vi "Main.vi"(0 "Proto File Path":path[](array[path]), 1 "Generated Library Name":string, 2 "Generate Server or Client?":enum16{"gRPC Server", "gRPC Client", "Both"}(ring), 3 "type of dialog (OK msg:1)":T1=1 items=["no dialog", "OK message", "continue or stop message", "OK message + warnings", "continue/stop + warnings"], 5 "Import Paths":path[](array[path]), 7 "Prototype Library":path, 9 "Target Project":path, 11 "Target Name":string, 12 "Library Suffix":string caption="Generated Library Suffix (\"_server\" / \"_client\" will be added by default)") -> (15 "error out":errorcluster)   [LabVIEW 2019, in "gRPC Template Creation Utility.lvlib"]
uses:
  gRPC Template Creation Utility.lvlib
  <vilib>/Utility/error.llb/DialogType.ctl
  TypeDefs/Project Settings.ctl
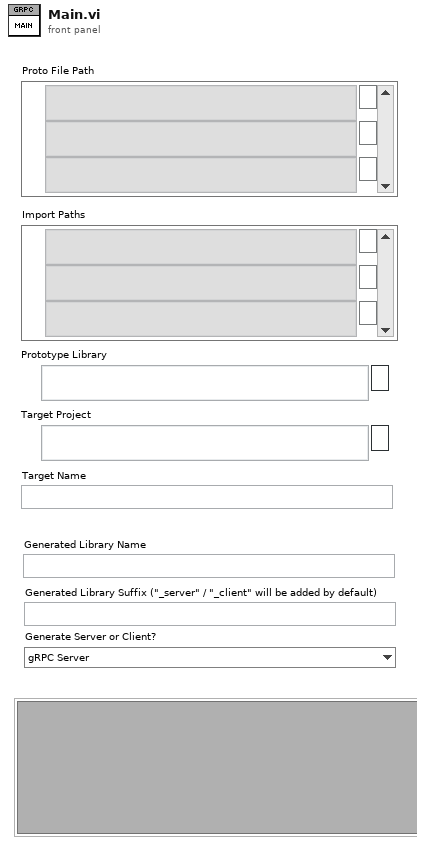
[diagram p1: front panel]
types:
  T1 = typedef "DialogType.ctl" = u16
  T2 = typedef "gRPC Template Creation Utility.lvlib/RPC Method Parameters.ctl" = cluster{"RPC Method Name":string, "Request Metadata Name":string, "Response Metadata Name":string, "Client Streaming":bool, "Server Streaming":bool}
  T3 = typedef "gRPC Template Creation Utility.lvlib/Enum Metadata (Scripting).ctl" = cluster{"Version":i32, "Name":string, "Type Url":string, "Enum Values":string, "Allow Alias":bool}
  T4 = typedef "gRPC Template Creation Utility.lvlib/Message Metadata (Scripting).ctl" = cluster{"Version":i32, "Name":string, "Type Url":string, "Elements":T5[], "Has Oneof":bool}
  T5 = typedef "gRPC Template Creation Utility.lvlib/Message Element Metadata (Scripting).ctl" = cluster{"Field Name":string, "Embedded Message Name":string, "Protobuf Index":i32, "MessageElementType":T6, "Repeated":bool, "Is in Oneof":bool, "Oneof Container Name":string}
  T6 = typedef "gRPC Template Creation Utility.lvlib/Message Element Type.ctl" = enum32{"Int32Value", "FloatValue", "DoubleValue", "BoolValue", "StringValue", "MessageValue", "Int64Value", "UInt32Value", "UInt64Value", "EnumValue", "Bytes", "Fixed64", "Fixed32", "SFixed64", "SFixed32", "SInt64", "SInt32"}
  T7 = typedef "gRPC Template Creation Utility.lvlib/Project Settings.ctl" = cluster{"Target Project Path":path, "Target Name":string, "Server Name":string, "Library Path":path}
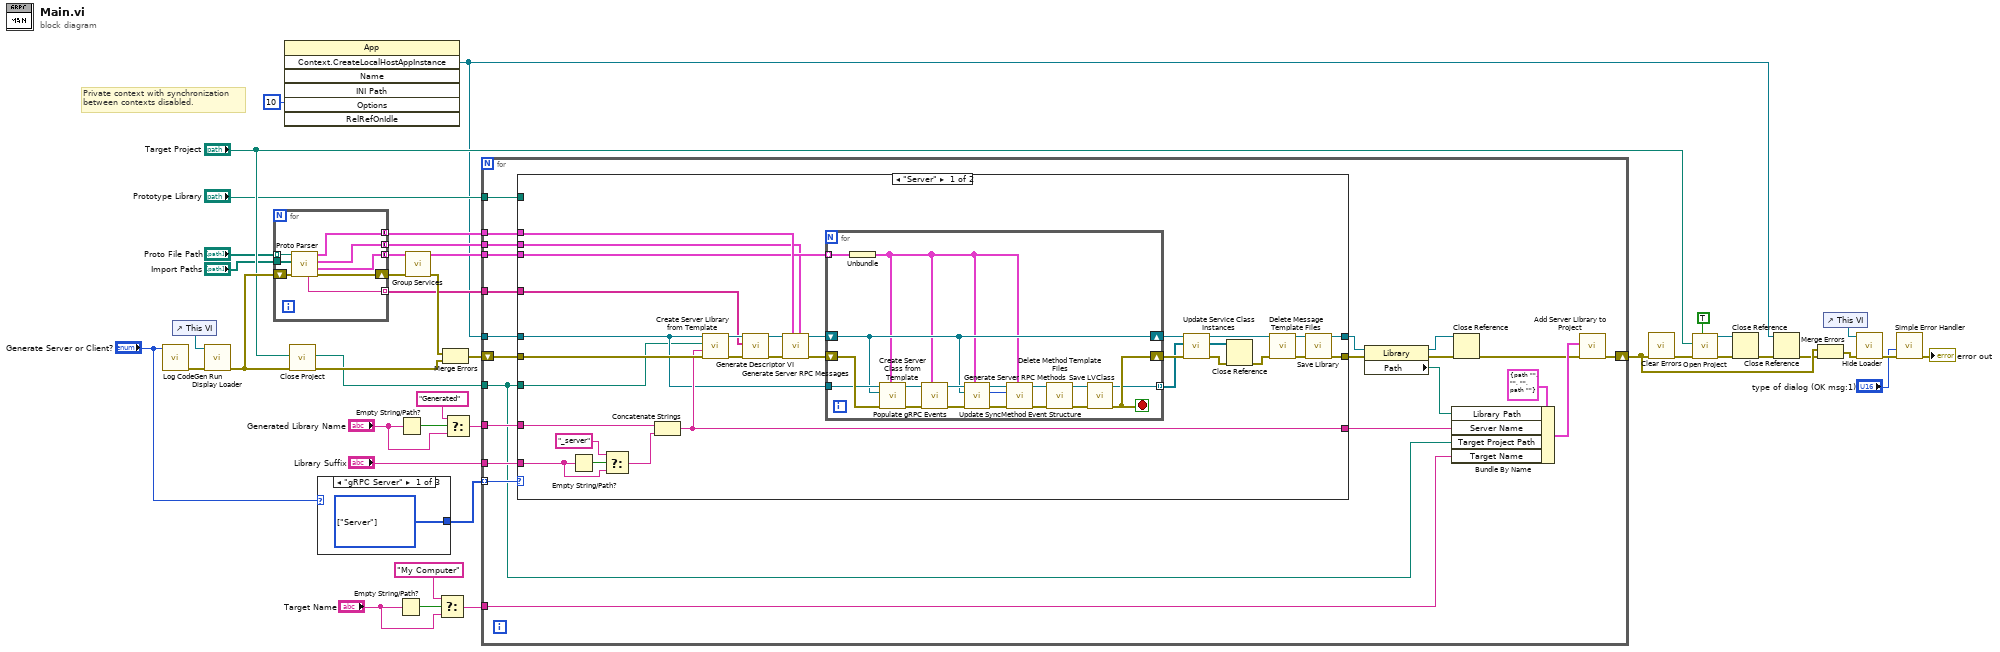
[diagram p0: block diagram]
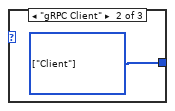
[diagram p2: hidden frame]
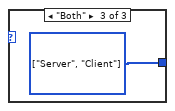
[diagram p3: hidden frame]
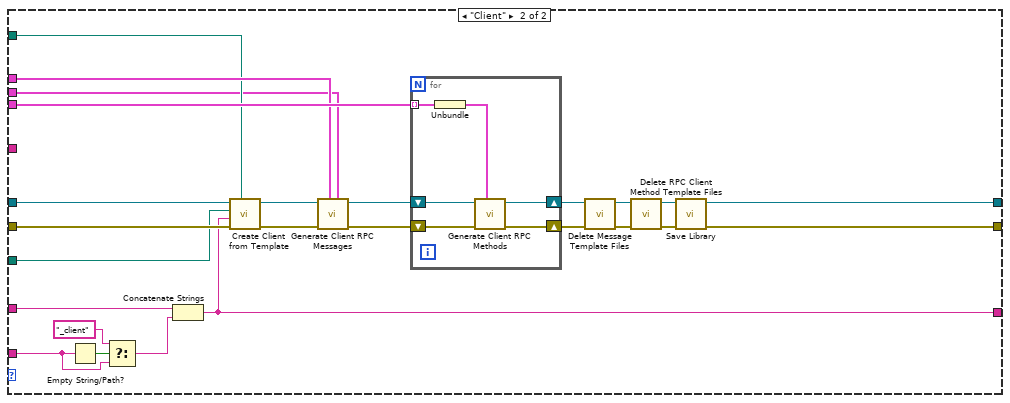
[diagram p4: hidden frame]
diagram:
  # "Private context with synchronization\nbetween contexts disabled."
  n1 = call "Log CodeGen Run.vi"("To Generate"="Generate Server or Client?") -> ("error out"=w8:errorcluster)  [unwired: 10 in]
  n2 = control-ref of="This VI"() -> (w7:refnum<vi>)
  n3 = call "Display Loader.vi"("error in (no error)"=w8, "VI in"=w7) -> ("error out"=w35:errorcluster)  [unwired: 9 in]
  n4 = for {
    tunnel: [w45] -> w37 mode=concatenating
    tunnel: [w49] -> w16 mode=concatenating
    shift-right: [w50] -> w18
    shift-left: w35 -> [w48]
    tunnel: "Proto File Path" -> [w47] mode=indexing
    tunnel: "Import Paths" -> [w46]
    tunnel: [w44] -> w11 mode=concatenating
    tunnel: [w43] -> w10 mode=indexing
    n5 = call "Proto Parser.vi"("error in (no error)"=w48, "Import Paths"=w46, ".proto file path"=w47) -> ("error out"=w50:errorcluster, "gRPC Method Parameters"=w49:T2[], "gRPC Enum Parameters"=w44:T3[], "gRPC Message Parameters"=w45:T4[], "Serialized Proto"=w43:string)  [unwired: 4 in]
  }
  n6 = invoke class="App" method="Context.CreateLocalHostAppInstance"("Options"=10) -> ("Create Context"=w3:refnum<vi>)  [unwired: 6 in, 6 out]
  n7 = call "Close Project.vi"("error in (no error)"=w35, "Project Path in"="Target Project") -> ("error out"=w39:errorcluster, "Project Path out"=w33:path)  [unwired: 8 in]
  n8 = case shown="\"gRPC Server\"" "Generate Server or Client?" {
    tunnel: [w51 w52 w53] -> w27
    frame "gRPC Server" {
      w51 = enum16{"Server", "Client"}[] [enum."Server"] items=["Server", "Client"]
    }
    frame "gRPC Client" {
      w52 = enum16{"Server", "Client"}[] [enum."Client"] items=["Server", "Client"]
    }
    frame "Both" {
      w53 = enum16{"Server", "Client"}[] [enum."Server", enum."Client"] items=["Server", "Client"]
    }
  }
  n9 = Empty String/Path?(string/path="Target Name") -> (empty?=w30:bool)
  n10 = Empty String/Path?(string/path="Generated Library Name") -> (empty?=w42:bool)
  n11 = call "Group Services.vi"("error in"=w18, "gRPC Method Parameters"=w16) -> ("error out"=w17:errorcluster, "Service Methods"=w15:cluster{"gRPC Method Parameters":T2[]}[])  [unwired: 8 in]
  n12 = Select(t="My Computer" ("Path"), s=w30, f="Target Name") -> (s? t:f=w28:string)
  n13 = Merge Errors(w17, w39) -> (w38:errorcluster)
  n14 = Select(t="Generated" ("Path"), s=w42, f="Generated Library Name") -> (s? t:f=w32:string)
  n15 = for {
    tunnel: w37 -> [w74]
    tunnel: w15 -> [w73]
    tunnel: w33 -> [w58]
    tunnel: w32 -> [w66]
    tunnel: w28 -> [w57]
    tunnel: w3 -> [w64]
    shift-right: [w61] -> w20
    shift-left: w38 -> [w75]
    tunnel: w27 -> [w60] mode=indexing
    tunnel: "Library Suffix" -> [w59]
    tunnel: "Prototype Library" -> [w56]
    tunnel: w11 -> [w55]
    tunnel: w10 -> [w54]
    n16 = case shown="\"Server\"" w60 {
      tunnel: w75 -> [w105 w148]
      tunnel: w74 -> [w104 w139]
      tunnel: w73 -> [w103 w147]
      tunnel: [w102 w146] -> w72
      tunnel: [w90 w138] -> w70
      tunnel: w66 -> [w101 w145]
      tunnel: [w100 w144] -> w65
      tunnel: w64 -> [w99 w143]
      tunnel: w58 -> [w98 w142]
      tunnel: w59 -> [w91 w133]
      tunnel: w56 -> [_ w131]
      tunnel: w55 -> [w83 w126]
      tunnel: w54 -> [w84 _]
      frame "Server" {
        n17 = Empty String/Path?(string/path=w91) -> (empty?=w94:bool)
        n18 = Select(t="_server" ("string"), s=w94, f=w91) -> (s? t:f=w92:string)
        n19 = Concatenate Strings(w101, w92) -> (w100:string)
        n20 = call "Create Server Library from Template.vi"("error in (no error)"=w105, "Generated Server Name"=w100, "Target Project Path"=w98, "Application ref in"=w99) -> ("error out"=w88:errorcluster, "Server library"=w86:refnum<vi>)  [unwired: 6 in]
        n21 = call "Generate Descriptor VI.vi"("error in (no error)"=w88, "Descriptor Strings"=w84, "Library in"=w86) -> ("error out"=w87:errorcluster, "Library out"=w85:refnum<vi>)  [unwired: 7 in]
        n22 = call "Generate Server RPC Messages.vi"("Enum Metadata"=w83, "Messages Metadata"=w104, "error in (no error)"=w87, "Library in"=w85) -> ("error out"=w89:errorcluster, "Library out"=w97:refnum<vi>)  [unwired: 6 in]
        n23 = for {
          tunnel: w103 -> [w121] mode=indexing
          shift-right: [w116] -> w81
          shift-left: w97 -> [w116]
          tunnel: w99 -> [w122]
          shift-right: [w108] -> w82
          shift-left: w89 -> [w123]
          tunnel: [w107] -> w79 mode=indexing
          stop <- w108 stop-if-true
          n24 = Unbundle(w121) -> ("gRPC Method Parameters"=w110:T2[])
          n25 = call "Create Server Class from Template.vi"("gRPC Method Parameters"=w110, "error in (no error)"=w123, "Library"=w116, "Application ref in"=w122) -> ("error out"=w119:errorcluster, "LVClassLibrary"=w120:refnum<vi>)  [unwired: 5 in, 1 out]
          n26 = call "Populate gRPC Events.vi"("RPC Method Parameters"=w110, "error in (no error)"=w119, "Server class in"=w120) -> ("error out"=w117:errorcluster, "Server class out"=w118:refnum<vi>)  [unwired: 7 in]
          n27 = call "Generate Server RPC Methods.vi"("RPC Method Parameters"=w110, "error in (no error)"=w117, "Library"=w116, "Server class in"=w118) -> ("error out"=w113:errorcluster, "Newly created methods count"=w109:i64, "Server class out"=w115:refnum<vi>)  [unwired: 5 in]
          n28 = call "Update SyncMethod Event Structure.vi"("gRPC Method Parameters"=w110, "error in (no error)"=w113, "Newly created methods count"=w109, "Server class in"=w115) -> ("error out"=w112:errorcluster, "Server class out"=w114:refnum<vi>)  [unwired: 6 in]
          n29 = call "Delete Method Template Files.vi"("error in (no error)"=w112, "LVClassLibrary in"=w114) -> ("error out"=w106:errorcluster, "LVClassLibrary out"=w111:refnum<vi>)  [unwired: 8 in]
          n30 = call "Save LVClass.vi"("error in (no error)"=w106, "LVClassLibrary in"=w111) -> ("error out"=w108:errorcluster, "LVClassLibrary out"=w107:refnum<vi>)  [unwired: 8 in]
        }
        n31 = call "Update Service Class Instances.vi"("error in (no error)"=w82, "service classes in"=w79, "server library in"=w81) -> ("error out"=w78:errorcluster, "service classes out"=w76:refnum<vi>[], "server library out"=w80:refnum<vi>)  [unwired: 6 in]
        n32 = Close Reference(reference=w76, error in (no error)=w78) -> (error out=w77:errorcluster)
        n33 = call "Delete Message Template Files.vi"("error in (no error)"=w77, "library in"=w80) -> ("error out"=w96:errorcluster, "library out"=w95:refnum<vi>)  [unwired: 8 in]
        n34 = call "Save Library.vi"("error in (no error)"=w96, "Library in"=w95) -> ("error out"=w90:errorcluster, "Library out"=w102:refnum<vi>)  [unwired: 8 in]
      }
      frame "Client" {
        n35 = Empty String/Path?(string/path=w133) -> (empty?=w135:bool)
        n36 = Select(t="_client" ("string"), s=w135, f=w133) -> (s? t:f=w132:string)
        n37 = Concatenate Strings(w145, w132) -> (w144:string)
        n38 = call "Create Client from Template.vi"("Template Library"=w131, "error in (no error)"=w148, "Generated Server Name"=w144, "Target Project Path"=w142, "Application ref in"=w143) -> ("error out"=w141:errorcluster, "Client library out"=w140:refnum<vi>)  [unwired: 5 in]
        n39 = call "Generate Client RPC Messages.vi"("Enum Metadata"=w126, "Messages Metadata"=w139, "error in (no error)"=w141, "Library in"=w140) -> ("error out"=w125:errorcluster, "Library out"=w124:refnum<vi>)  [unwired: 6 in]
        n40 = for {
          tunnel: w147 -> [w154] mode=indexing
          shift-right: [w149] -> w129
          shift-left: w124 -> [w151]
          shift-right: [w150] -> w130
          shift-left: w125 -> [w152]
          n41 = Unbundle(w154) -> ("gRPC Method Parameters"=w153:T2[])
          n42 = call "Generate Client RPC Methods.vi"("rpc method parameters"=w153, "error in (no error)"=w152, "library in"=w151) -> ("error out"=w150:errorcluster, "library out"=w149:refnum<vi>)  [unwired: 7 in]
        }
        n43 = call "Delete Message Template Files.vi"("error in (no error)"=w130, "library in"=w129) -> ("error out"=w127:errorcluster, "library out"=w128:refnum<vi>)  [unwired: 8 in]
        n44 = call "Delete RPC Client Method Template Files.vi"("error in (no error)"=w127, "library in"=w128) -> ("error out"=w136:errorcluster, "library out"=w137:refnum<vi>)  [unwired: 8 in]
        n45 = call "Save Library.vi"("error in (no error)"=w136, "Library in"=w137) -> ("error out"=w138:errorcluster, "Library out"=w146:refnum<vi>)  [unwired: 8 in]
      }
    }
    n46 = property class="Library"(reference=w72, error in=w70) -> (reference out=w71:refnum<vi>, error out=w63:errorcluster, "Path"=w68:path)
    n47 = Bundle By Name(cluster=T7 {"Target Project Path"=path "", "Target Name"="", "Server Name"="", "Library Path"=path ""} ("Project Settings"), "Library Path"=w68, "Server Name"=w65, "Target Project Path"=w58, "Target Name"=w57) -> (w67:T7)
    n48 = Close Reference(reference=w71, error in (no error)=w63) -> (error out=w62:errorcluster)
    n49 = call "Add Server Library to Project.vi"("error in (no error)"=w62, "Project Settings"=w67) -> ("error out"=w61:errorcluster)  [unwired: 9 in]
  }
  n50 = call <vilib>:"Clear Errors.vi"("error in (no error)"=w20) -> ("error out"=w22:errorcluster)  [unwired: 5 in, 1 out]
  n51 = call "Open Project.vi"("Open Project Window ?"=TRUE, "error in (no error)"=w22, "Project Path in"="Target Project") -> ("error out"=w24:errorcluster, "Project out"=w25:refnum<vi>)  [unwired: 7 in]
  n52 = Close Reference(reference=w25, error in (no error)=w24) -> (error out=w5:errorcluster)
  n53 = Close Reference(reference=w3, error in (no error)=w5) -> (error out=w4:errorcluster)
  n54 = Merge Errors(w20, w4) -> (w21:errorcluster)
  n55 = control-ref of="This VI"() -> (w36:refnum<vi>)
  n56 = call "Hide Loader.vi"("error in (no error)"=w21, "VI in"=w36) -> ("error out"=w34:errorcluster)  [unwired: 9 in]
  n57 = call <vilib>:"Simple Error Handler.vi"("type of dialog (OK msg:1)"="type of dialog (OK msg:1)", "error in (no error)"=w34) -> ("error out"=→"error out":errorcluster)  [unwired: 3 in, 4 out]
